vi "Sauvegarde distant.vi"() -> ()   [LabVIEW 2022 SP3]
uses:
  Variables globales/Variable glob generale.vi
panel:
  out "Chemin du fichier de sauvegarde :":path
  out "Dossier fichier sauvegarde":path
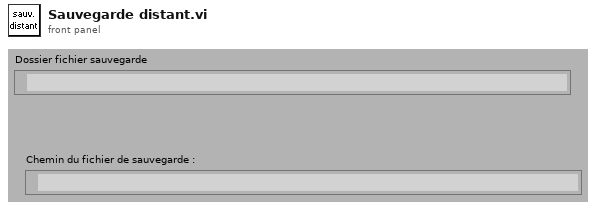
[diagram p1: front panel]
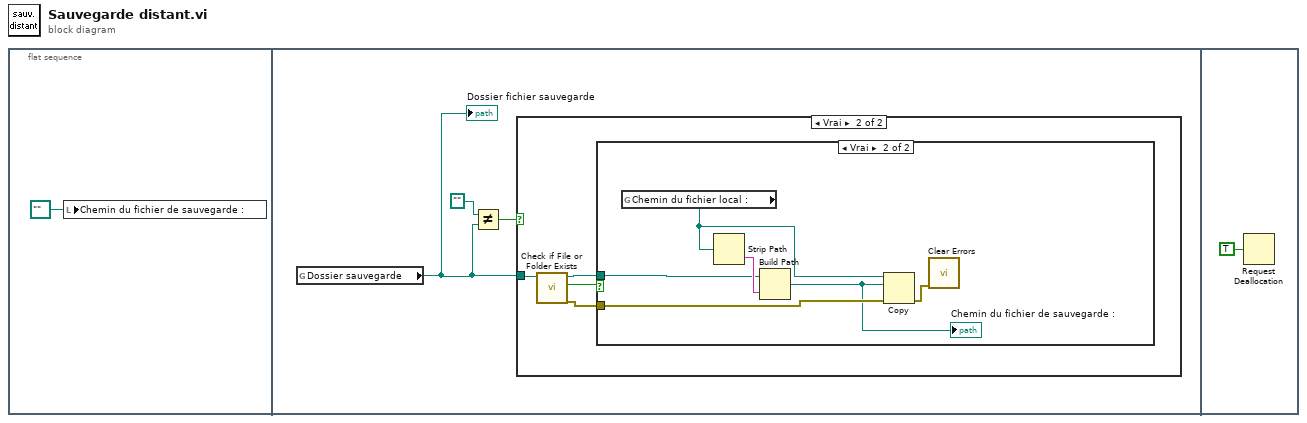
[diagram p0: block diagram]
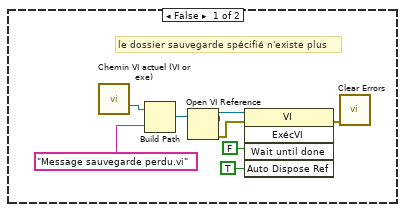
[diagram p3: hidden frame]
diagram:
  n1 = flat-sequence {
    frame #0 {
      n2 = local write "Chemin du fichier de sauvegarde :"(path "" ("Chemin du fichier distant :")) -> ()
    }
    frame #1 {
      n3 = global read "Variable glob generale.vi" "Dossier sauvegarde"() -> (w3:path)
      "Dossier fichier sauvegarde" <- w3
      n4 = Not Equal?(x=path "", y=w3) -> (x != y?=w2:bool)
      n5 = case shown="Vrai" w2 {
        tunnel: w3 -> [_ w8]
        frame False {
        }
        frame True {
          n6 = call <vilib>:"Check if File or Folder Exists.vi"("path"=w8) -> ("error out"=w5:errorcluster, "file or folder exists?"=w6:bool, "dup path"=w7:path)  [unwired: 8 in]
          n7 = case shown="Vrai" w6 {
            tunnel: w7 -> [_ w21]
            tunnel: w5 -> [_ w20]
            frame False {
              # "le dossier sauvegarde spécifié n'existe plus"
              n8 = call "Chemin VI actuel (VI or exe).vi"() -> ("VI or executable installation directory"=w10:path)  [unwired: 14 in, 1 out]
              n9 = Build Path(base path=w10, name or relative path="Message sauvegarde perdu.vi" ("nom ou chemin relatif")) -> (appended path=w15:path)
              n10 = Open VI Reference(vi path=w15) -> (vi reference=w13:refnum<vi>, error out=w12:errorcluster)  [unwired: 5 in]
              n11 = invoke class="VI" method="ExécVI"(reference=w13, error in=w12, "Wait until done"=FALSE ("Attendre la fin"), "Auto Dispose Ref"=TRUE ("Supprimer la référence automatiquement")) -> (error out=w11:errorcluster)  [unwired: 1 in, 4 out]
              n12 = call <vilib>:"Clear Errors.vi"("error in (no error)"=w11) -> ()  [unwired: 5 in, 2 out]
            }
            frame True {
              n13 = global read "Variable glob generale.vi" "Chemin du fichier local :"() -> (w17:path)
              n14 = Strip Path(path=w17) -> (name=w22:string)  [unwired: 1 out]
              n15 = Build Path(base path=w21, name or relative path=w22) -> (appended path=w18:path)
              "Chemin du fichier de sauvegarde :" <- w18
              n16 = Copy(8:w20, 10:w18, 11:w17) -> (0:w19:errorcluster)  [unwired: 2 in, 2 out]
              n17 = call <vilib>:"Clear Errors.vi"("error in (no error)"=w19) -> ()  [unwired: 5 in, 2 out]
            }
          }
        }
      }
    }
    frame #2 {
      n18 = Request Deallocation(TRUE ("flag")) -> ()
    }
  }
